vi "publishJobReport.vi"(8 "error in (no error)":errorcluster, 11 "Job in":refnum<class "Job.lvclass">) -> (0 "error out":errorcluster, 2 "JobReport":refnum<class "JobReport.lvclass">, 3 "Job out":refnum<class "Job.lvclass">)   [LabVIEW 2013, in "openCronJob.lvlib" / "Job.lvclass"]
uses:
  Job.lvclass
  JobReport/JobReport.lvclass
  Job.lvclass/Job.ctl
  JobReport/JobReport.lvclass/JobReport.ctl
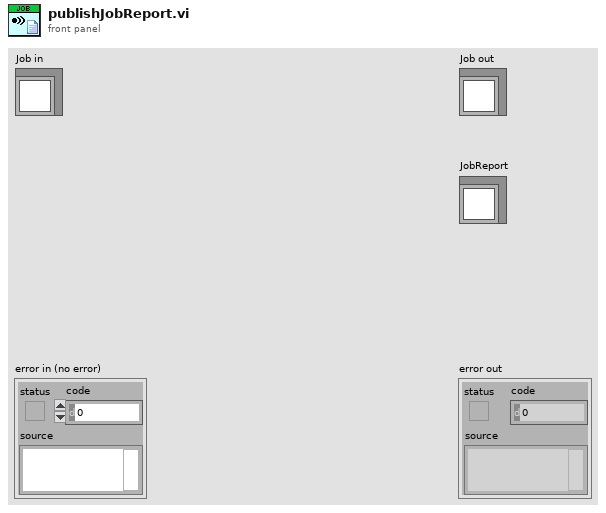
[diagram p1: front panel]
types:
  T1 = typedef "openCronJob.lvlib/JobReport.lvclass/Job Report -- cluster.ctl" = cluster{"Name":string, "GUID":string, "Start Time":timestamp, "Duration (s)":dbl, "exception code":i32, "stdin":string, "stdout":string}
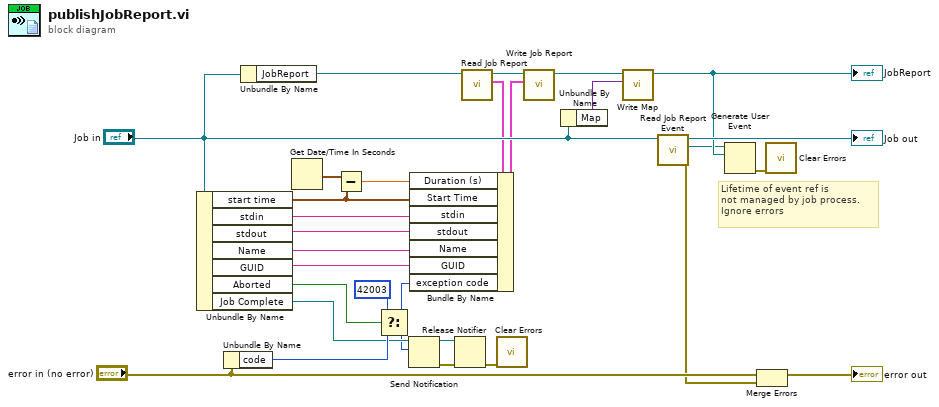
[diagram p0: block diagram]
diagram:
  # "Lifetime of event ref is\nnot managed by job process. \nIgnore errors"
  n1 = Unbundle By Name("Job in") -> ("start time"=w21:timestamp, "stdin"=w15:string, "stdout"=w14:string, "Name"=w24:string, "GUID"=w23:string, "Aborted"=w17:bool, "Job Complete"=w12:refnum<notifier>)
  n2 = Unbundle By Name("error in (no error)") -> ("code"=w13:i32)
  n3 = Unbundle By Name("Job in") -> ("JobReport"=w2:refnum<class "JobReport.lvclass">)
  n4 = Get Date/Time In Seconds() -> (seconds since 1Jan1904=w22:timestamp)
  n5 = Subtract(x=w22, y=w21) -> (x-y=w20:dbl)
  n6 = Select(t=42003, s=w17, f=w13) -> (s? t:f=w11:i32)
  n7 = Send Notification(notification=w11, notifier=w12) -> (notifier out=w9:refnum<notifier>, error out=w8:errorcluster)  [unwired: 1 in]
  n8 = Release Notifier(notifier=w9, error in (no error)=w8) -> (error out=w10:errorcluster)  [unwired: 1 in, 2 out]
  n9 = call "Read Job Report.vi"("JobReport in"=w2) -> ("Job Report"=w7:T1, "JobReport out"=w6:refnum<class "JobReport.lvclass">)  [unwired: 8 in, 1 out]
  n10 = Bundle By Name(cluster=w7, "Duration (s)"=w20, "Start Time"=w21, "stdin"=w15, "stdout"=w14, "Name"=w24, "GUID"=w23, "exception code"=w11) -> (w1:T1)
  n11 = call <vilib>:"Clear Errors.vi"("error in (no error)"=w10) -> ()  [unwired: 6 in, 1 out]
  n12 = call "Write Job Report.vi"("Job Report"=w1, "JobReport in"=w6) -> ("JobReport out"=w5:refnum<class "JobReport.lvclass">)  [unwired: 8 in, 1 out]
  n13 = Unbundle By Name("Job in") -> ("Map"=w4:variant)
  n14 = call "Write Map.vi"("Map"=w4, "JobReport in"=w5) -> ("JobReport out"=w25:refnum<class "JobReport.lvclass">)  [unwired: 8 in, 1 out]
  "JobReport" <- w25
  n15 = call "Read Job Report Event.vi"("Job in"="Job in") -> ("error out"=w3:errorcluster, "Job Report Event"=w18:refnum<user-event>, "Job out"=→"Job out":refnum<class "Job.lvclass">)  [unwired: 6 in, 2 out]
  n16 = Generate User Event(user event=w18, event data cluster=w25) -> (error out=w19:errorcluster)  [unwired: 2 in, 1 out]
  n17 = Merge Errors("error in (no error)", w3) -> (→"error out":errorcluster)
  n18 = call <vilib>:"Clear Errors.vi"("error in (no error)"=w19) -> ()  [unwired: 6 in, 1 out]
